vi "Calibration - SubVI.vi"() -> (1 "Interpolation Method":T1, 3 "Distance [cm] | Voltage [V]":dbl[][](array[numeric]))   [LabVIEW 2025]
uses:
  Interpolation_Method.ctl
  <vilib>/Utility/file.llb/Read Delimited Spreadsheet (DBL).vi
  <vilib>/Utility/file.llb/Write Delimited Spreadsheet (DBL).vi
  <vilib>/gmath/NI_Gmath.lvlib
panel:
  in  "Interpolation Method":T1
  out "XY Graph":T2(graph)
  in  "Distance [cm] | Voltage [V]":dbl[][](array[numeric])
  in  "Reset graph":bool
  in  "Finish Calibration (Return to main)":bool
  in  "Start calibration":bool
  in  "Save calibration file":bool
  in  "Import calibration file":bool
  # "Calibration table"
  # "Write calibration data to array or import from file"
  # "Exported calibration data"
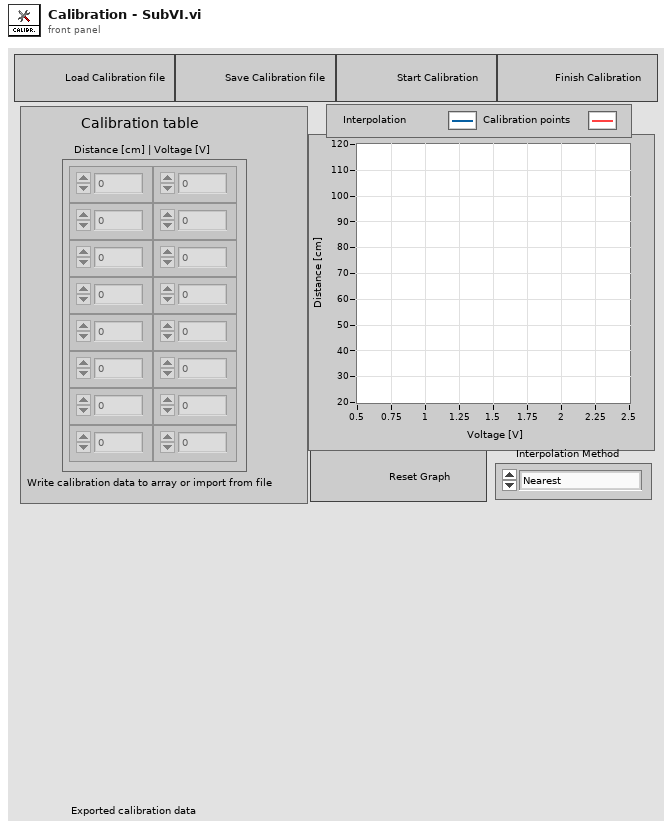
[diagram p1: front panel]
types:
  T1 = typedef "Interpolation_Method.ctl" = enum16{"Nearest", "Linear", "Spline", "Cubic Hermite", "Lagrange"}
  T2 = cluster{"Distance [cm] | Voltage [V]":dbl[], "Distance [cm] | Voltage [V]":dbl[]}[]
  T3 = cluster{"Distance [cm] | Voltage [V]":dbl[], "Distance [cm] | Voltage [V]":dbl[]}
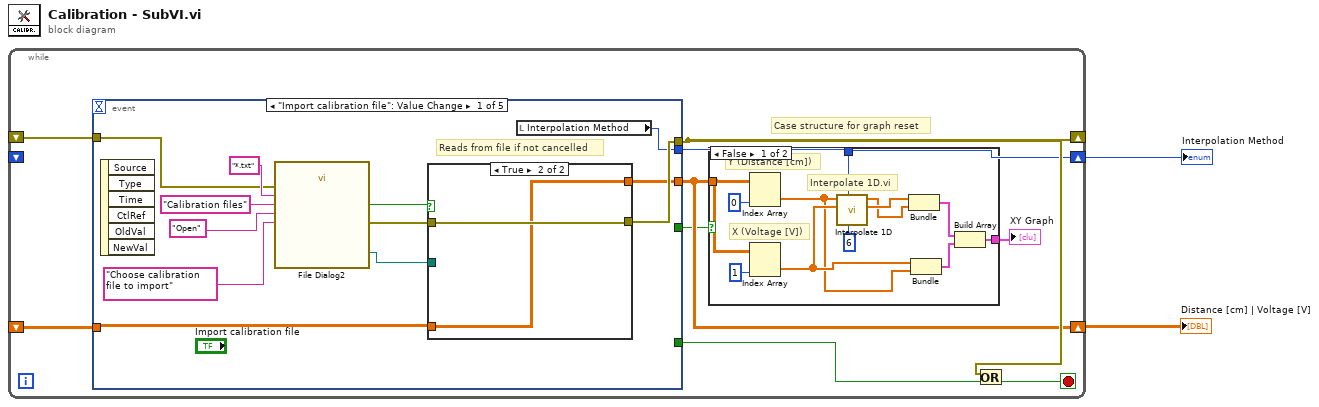
[diagram p0: block diagram]
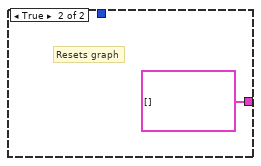
[diagram p2: hidden frame]
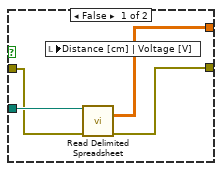
[diagram p3: hidden frame]
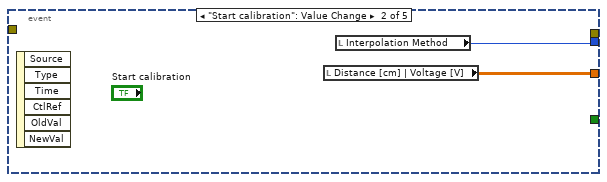
[diagram p4: hidden frame]
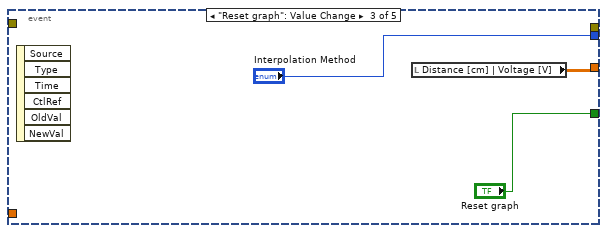
[diagram p5: hidden frame]
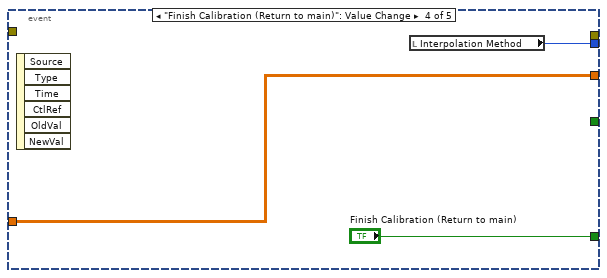
[diagram p6: hidden frame]
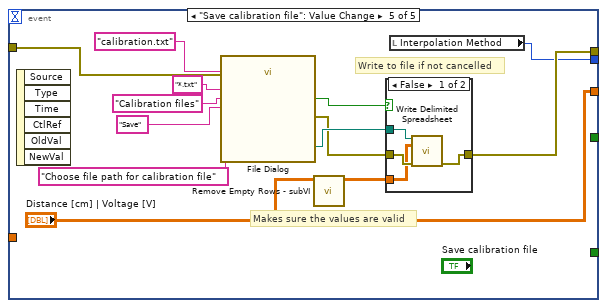
[diagram p7: hidden frame]
diagram:
  n1 = while {
    shift-right: [w7] -> _
    shift-left: _ -> [w11]
    shift-right: [w6] -> w2
    shift-left: _ -> [w5]
    shift-right: [w4] -> w1
    shift-left: _ -> [_]
    stop <- w9 stop-if-true
    # "Case structure for graph reset"
    n2 = event shown="[0] \"Import calibration file\": Value Change" {
      selector: _ -> [_ _ _ _ _]
      dyn-events: _ -> [_ _ _ _ _]
      timeout: _ -> [_ _ _ _ _]
      tunnel: [w29 _ _ _ w55] -> w7
      tunnel: w11 -> [w32 _ _ _ w62]
      tunnel: [w27 w44 w46 w49 "Distance [cm] | Voltage [V]"] -> w6
      tunnel: [w26 w43 "Interpolation Method" w48 w51] -> w4
      tunnel: [_ _ _ "Finish Calibration (Return to main)" _] -> w8
      tunnel: w5 -> [w25 _ _ w49 _]
      tunnel: [_ _ "Reset graph" _ _] -> w3
      event "Import calibration file": Value Change {
        # "Reads from file if not cancelled"
        n3 = event-data() -> ()  [unwired: 1 in, 6 out]
        n4 = call "File Dialog2"("prompt"="Choose calibration file to import", "button label"="Open", "error in"=w32, "pattern (all files)"="*.txt", "pattern label"="Calibration files") -> ("selected path"=w28:path, "cancelled"=w31:bool, "error out"=w30:errorcluster)  [unwired: 7 in, 1 out]
        n5 = case shown="True" w31 {
          tunnel: w30 -> [w39 w42]
          tunnel: [w38 w42] -> w29
          tunnel: w28 -> [w40 _]
          tunnel: [w37 w41] -> w27
          tunnel: w25 -> [_ w41]
          frame False {
            n6 = call-poly <vilib>:"Read Delimited Spreadsheet.vi"("file path (dialog if empty)"=w40, "error in (no error)"=w39) -> ("all rows"=w37:dbl[][], "error out"=w38:errorcluster)  [unwired: 8 in, 4 out]
            n7 = local write "Distance [cm] | Voltage [V]"(w37) -> ()
          }
          frame True {
          }
        }
        n8 = local read "Interpolation Method"() -> (w26:T1)
      }
      event "Start calibration": Value Change {
        n9 = event-data() -> ()  [unwired: 1 in, 6 out]
        n10 = local read "Distance [cm] | Voltage [V]"() -> (w44:dbl[][])
        n11 = local read "Interpolation Method"() -> (w43:T1)
      }
      event "Reset graph": Value Change {
        n12 = event-data() -> ()  [unwired: 1 in, 6 out]
        n13 = local read "Distance [cm] | Voltage [V]"() -> (w46:dbl[][])
      }
      event "Finish Calibration (Return to main)": Value Change {
        n14 = event-data() -> ()  [unwired: 1 in, 6 out]
        n15 = local read "Interpolation Method"() -> (w48:T1)
      }
      event "Save calibration file": Value Change {
        # "Makes sure the values are valid"
        # "Write to file if not cancelled"
        n16 = event-data() -> ()  [unwired: 1 in, 6 out]
        n17 = call "File Dialog"("prompt"="Choose file path for calibration file", "button label"="Save", "default name"="calibration.txt", "error in"=w62, "pattern (all files)"="*.txt", "pattern label"="Calibration files") -> ("selected path"=w57:path, "cancelled"=w54:bool, "error out"=w56:errorcluster)  [unwired: 6 in, 1 out]
        n18 = call "Remove Empty Rows - subVI.vi"("Distance [cm] | Voltage [V]"="Distance [cm] | Voltage [V]") -> ("Valid calibration points"=w53:dbl[][])  [unwired: 10 in]
        n19 = case shown="False" w54 {
          tunnel: w57 -> [w67 _]
          tunnel: w56 -> [w66 w68]
          tunnel: [w65 w68] -> w55
          tunnel: w53 -> [w64 _]
          frame False {
            n20 = call-poly <vilib>:"Write Delimited Spreadsheet.vi"("file path (dialog if empty)"=w67, "2D data"=w64, "error in (no error)"=w66) -> ("error out"=w65:errorcluster)  [unwired: 11 in, 1 out]
          }
          frame True {
          }
        }
        n21 = local read "Interpolation Method"() -> (w51:T1)
      }
    }
    n22 = case shown="False" w3 {
      tunnel: [w14 T2 []] -> w10
      tunnel: w6 -> [w13 _]
      tunnel: w4 -> [w12 _]
      frame False {
        # "Interpolate 1D.vi"
        # "X (Voltage [V])"
        # "Y (Distance [cm])"
        n23 = Index Array(array=w13, index (col)=0 ("disabled index (col)")) -> (element=w17:dbl[])  [unwired: 1 in]
        n24 = Index Array(array=w13, index (col)=1 ("disabled index (col)")) -> (element=w18:dbl[])  [unwired: 1 in]
        n25 = call <vilib>:"Interpolate 1D.vi"("ntimes"=6, "method"=w12, "X"=w18, "Y"=w17) -> ("xi used"=w20:dbl[], "yi"=w19:dbl[])  [unwired: 5 in, 1 out]
        n26 = Bundle("xi used"=w20, "yi"=w19) -> (w15:cluster{"xi used":dbl[], "yi":dbl[]})  [unwired: 1 in]
        n27 = Bundle("Distance [cm] | Voltage [V]"=w18, "Distance [cm] | Voltage [V]"=w17) -> (w16:T3)  [unwired: 1 in]
        n28 = Build Array(w15, w16) -> (w14:T2)
      }
      frame True {
        # "Resets graph"
      }
    }
    "XY Graph" <- w10
    n29 = Or(x=w7, y=w8) -> (x .or. y?=w9:bool)
  }
  "Distance [cm] | Voltage [V]" <- w2
  "Interpolation Method" <- w1
